vi "Test Plugin Requirements.vi"() -> (0 "error out":errorcluster)   [LabVIEW 2026]
doc: "PLG-ROLE-001: required Standard Measurement hardware roles are exact and ordered."
uses:
  source/plugins/measurements/Standard Measurement Plugin/Standard Measurement.lvclass
  <vilib>/addons/_JKI Toolkits/Caraya/classes/Test/Test.lvclass
  <vilib>/addons/_JKI Toolkits/Caraya/classes/Assert/Assert.lvclass
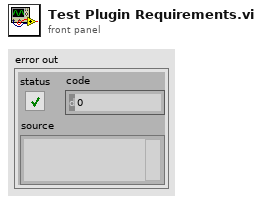
[diagram p1: front panel]
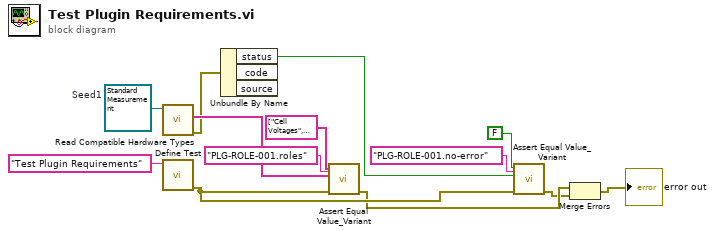
[diagram p0: block diagram]
diagram:
  w12 = refnum<class "Standard Measurement.lvclass"> refnum  # Seed1
  n1 = call-dynamic "Read Compatible Hardware Types.vi"("Standard Measurement in"=w12) -> ("error out"=w8:errorcluster, "Compatible Hardware Types"=w9:string[])  [unwired: 8 in, 1 out]
  n2 = call <vilib>:"Define Test.vi"("Label (VI Title)"="Test Plugin Requirements") -> ("error out"=w4:errorcluster)  [unwired: 9 in, 1 out]
  n3 = Unbundle By Name(w8) -> ("status"=w5:bool)  [unwired: 2 out]
  n4 = call <vilib>:"Assert Equal Value_Variant.vi"("Label"="PLG-ROLE-001.roles", "error in (no error)"=w4, "Actual"=w9, "Expected"=string[] ["Cell Voltages", "Pack Temperatures", "Something Else"]) -> ("error out"=w3:errorcluster)  [unwired: 6 in, 1 out]
  n5 = call <vilib>:"Assert Equal Value_Variant.vi"("Label"="PLG-ROLE-001.no-error", "error in (no error)"=w4, "Actual"=w5, "Expected"=FALSE) -> ("error out"=w2:errorcluster)  [unwired: 6 in, 1 out]
  n6 = Merge Errors(w3, w2) -> (→"error out":errorcluster)
